vi "VIH HelpGen - HTML - Find Service Tag.vi"(8 "Offset in (0)":i32, 10 "Tag name":string, 11 "HTML in":string) -> (0 "Offset out":i32, 1 "After":string, 2 "Compete Tag":string, 3 "Before":string)   [LabVIEW 2014]
doc: "::: VI Helpeks :::\nCopyright (c) 2000-2026 Konstantin Shifershteyn. All rights reserved."
panel:
  # "VI Helpeks\nCopyright (c) 2012-2026 Konstantin Shifershteyn"
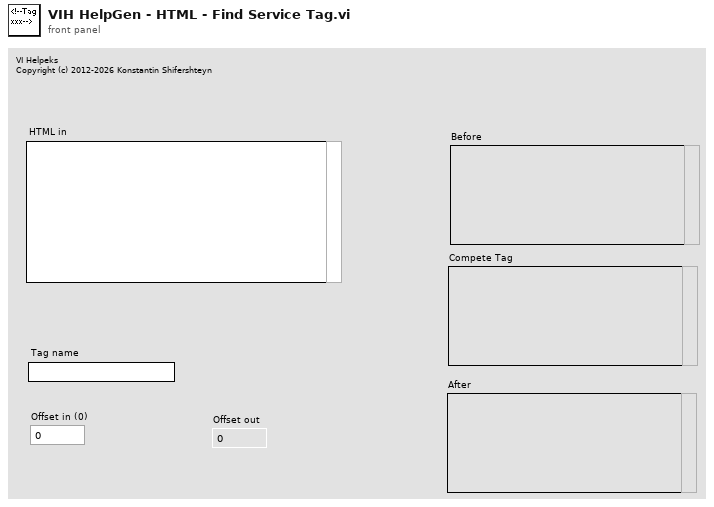
[diagram p1: front panel]
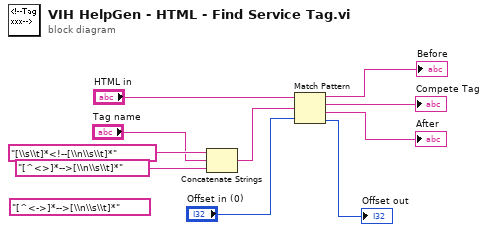
[diagram p0: block diagram]
diagram:
  (unwired) "[^<->]*-->[\\n\\s\\t]*"
  n1 = Concatenate Strings("[\\s\\t]*<!--[\\n\\s\\t]*", "Tag name", "[^<>]*-->[\\n\\s\\t]*") -> (w7:string)
  n2 = Match Pattern(string="HTML in", regular expression=w7, offset (0)="Offset in (0)") -> (before substring=→"Before":string, match substring=→"Compete Tag":string, after substring=→"After":string, offset past match=→"Offset out":i32)
